vi "串口读写 - WK.vi"(8 "错误输入（无错误）":errorcluster, 9 "是否保存?(F)":bool, 10 "写入设备":string, 11 "VISA输入":refnum<visa-resource-name>) -> (0 "错误输出":errorcluster, 1 "读取设备(n)":dbl format="%.2g", 2 "读取设备":string, 3 "VISA输出":refnum<visa-resource-name>)   [LabVIEW 2026, in "UI-温度控制.lvlib"]
uses:
  e88502f5-6bb7-421a-b420-d82910cf4c73.vi
  b8b55d77-a596-4c3d-9485-8cafcfd9cda6.vi
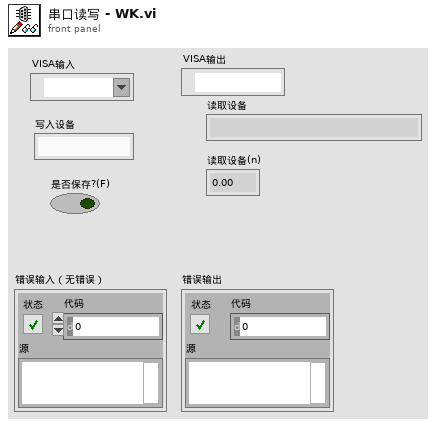
[diagram p1: front panel]
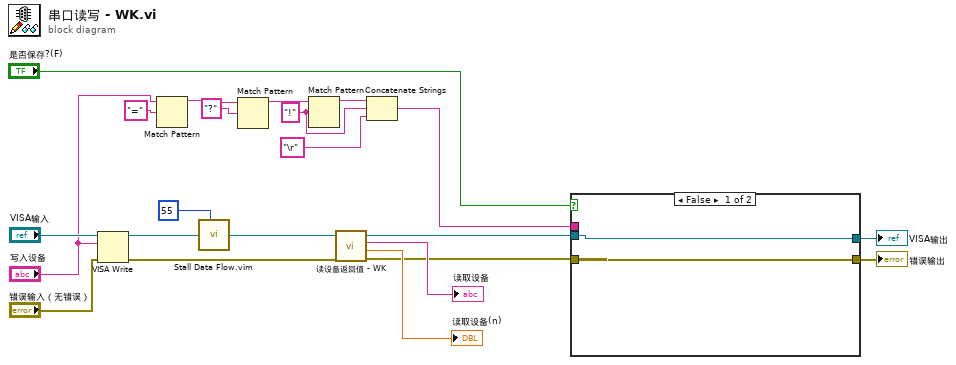
[diagram p0: block diagram]
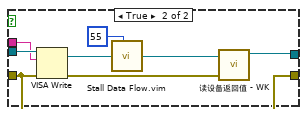
[diagram p2: hidden frame]
diagram:
  w6 = "!" ("正则表达式")
  n1 = VISA Write(VISA resource name="VISA输入", write buffer="写入设备", error in (no error)="错误输入（无错误）") -> (VISA resource name out=w20:refnum<visa-resource-name>, error out=w19:errorcluster)  [unwired: 1 out]
  n2 = Match Pattern(string="写入设备", regular expression="=" ("正则表达式")) -> (before substring=w9:string)  [unwired: 1 in, 3 out]
  n3 = call "Stall Data Flow.vim"("value in"=w20, "milliseconds to wait"=u32 55 ("等待时间（毫秒）")) -> ("value out"=w2:refnum<visa-resource-name>)  [unwired: 1 out]
  n4 = Match Pattern(string=w9, regular expression="?" ("正则表达式")) -> (before substring=w8:string)  [unwired: 1 in, 3 out]
  n5 = Match Pattern(string=w8, regular expression=w6) -> (before substring=w7:string)  [unwired: 1 in, 3 out]
  n6 = call "读设备返回值 - WK.vi"("错误输入（无错误）"=w19, "VISA引用句柄输入"=w2) -> ("错误输出"=w15:errorcluster, "读取设备(n)"=→"读取设备(n)":dbl, "读取设备"=→"读取设备":string, "VISA引用句柄输出"=w16:refnum<visa-resource-name>)  [unwired: 6 in]
  n7 = Concatenate Strings(w7, w6, "\r" ("写入缓冲区")) -> (w3:string)
  n8 = case shown="False" "是否保存?(F)" {
    tunnel: w16 -> [w24 w32]
    tunnel: w15 -> [w23 w27]
    tunnel: [w24 w28] -> w14
    tunnel: [w23 w27] -> w13
    tunnel: w3 -> [_ w29]
    frame False {
    }
    frame True {
      n9 = VISA Write(VISA resource name=w32, write buffer=w29, error in (no error)=w27) -> (VISA resource name out=w31:refnum<visa-resource-name>, error out=w30:errorcluster)  [unwired: 1 out]
      n10 = call "Stall Data Flow.vim"("value in"=w31, "milliseconds to wait"=u32 55) -> ("value out"=w26:refnum<visa-resource-name>)  [unwired: 1 out]
      n11 = call "读设备返回值 - WK.vi"("错误输入（无错误）"=w30, "VISA引用句柄输入"=w26) -> ("VISA引用句柄输出"=w28:refnum<visa-resource-name>)  [unwired: 6 in, 3 out]
    }
  }
  "VISA输出" <- w14
  "错误输出" <- w13
